vi "Two Color Calibration.vi"(7 "Calling VI Ref":refnum<vi>) -> ()   [LabVIEW 2016]
uses:
  <vilib>/Utility/miscctls.llb/LVPointTypeDef.ctl
  Hardware Configuration/Hardware Configuration Controls/Device Type.ctl
  Hardware Configuration/Hardware Configuration Controls/Device Function.ctl
  Two Color Cal Type Defs/Two Color Cal Notifier Type.ctl
  Two Color Cal Type Defs/Two Color Cal Actions.ctl
  Two Color Cal Type Defs/Two Color Last Used Parameters.ctl
  Orca Flash Capture Manager/SMS Analysis Interface/SMS Analysis Interface Type Defs/SMS Analysis Interface Connection Info.ctl
  Tools/TIFF Image Read and Write/ImageJ TIF Type Defs/TIF Write Image Information.ctl
  Device Library/Cameras/Camera Controls/Generic Camera Actions.ctl
  Laser Control/Laser Power Control/Laser Power Control Type Defs/Laser Power Ctrl Messenger Actions.ctl
  Device Library/Stages/Stages Controls/Stage Actions.ctl
  shell32.dll
panel:
  out "Transfer Error":bool
  in  "Auto Focus":bool
  in  "Auto Run":bool=TRUE
  out "File Close":errorcluster
  in  "Skip":bool
  in  "Run Capture":bool
  in  "Number of Y Steps":u16=10
  out "Current Y Step":u16
  out "Current X Step":u16
  in  "Number of X Steps":u16=10
  in  "Step Size (µm)":dbl=2.0
  in  "Start":bool
  in  "Quit":bool
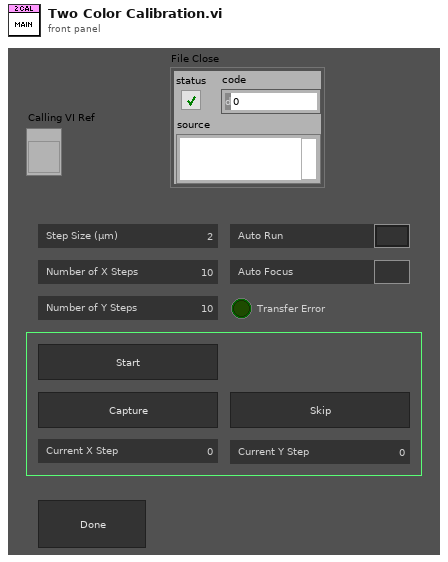
[diagram p1: front panel]
types:
  T1 = typedef "SMS Analysis Interface Connection Info.ctl" = cluster{"Remote IP":string, "Port":u16}
  T2 = typedef "Two Color Last Used Parameters.ctl" = cluster{"Step Size (um)":dbl, "No X Steps":u16, "No Y Steps":u16, "Auto Run":bool, "Auto Focus":bool}
  T3 = typedef "Device Function.ctl" = enum16{"Primary", "Secondary", "Overview", "Wide Field Drift Correction", "642 nm Excitation", "560 nm Excitation", "940 nm Excitation", "546 nm Excitation", "488 nm Excitation", "405 nm Excitation", "Objective Drift Correction", "4Pi Objective Lock", "Objective XY", "Objective Z", "Sample XY", "Sample Coarse Z", "Sample Z", "4Pi Lower", "4Pi Upper", "Mojo", "Adj Cavity", "Line Scanning", "Alert"}
  T4 = typedef "Device Type.ctl" = enum16{"AOTF", "Camera", "Deformable Mirror", "Laser", "Shutter", "Stage", "Waveform", "FPGA", "Email", "Filter Wheel"}
  T5 = typedef "Two Color Cal Actions.ctl" = enum16{"Idle", "Set File Name", "Open FIle", "Start Camera", "Laser On", "Auto Focus", "Capture", "Move XY", "Pause Scan", "Abort", "Send Image", "Quit"}
  T6 = typedef "Two Color Cal Notifier Type.ctl" = cluster{"Actions":T5, "X Steps":u16, "Y Steps":u16, "Save File Path":path, "Save File Ref":refnum<file>}
  T7 = enum16{"Always On", "Always Off", "Off While Running"}
  T8 = typedef "LVPointTypeDef.ctl" = cluster{"Horizontal":i16, "Vertical":i16}
  T9 = typedef "Generic Camera Actions.ctl" = enum16{"Status", "Live Preview", "Capture", "Abort", "Set Exposure Time (s)", "Get Exposure Time (s)", "Record Settings", "Binning", "Set ROI", "Get ROI", "Defect Correction On?", "Cooler On?", "Fan On?", "Quit"}
  T10 = typedef "TIF Write Image Information.ctl" = cluster{"Image Width (Pixels)":u32, "Image Height (Pixels)":u32, "Pixel Width (µm)":dbl, "Pixel Height (µm)":dbl, "Bits Per Sample (e.g. 16)":u32, "No. of Frames":u32, "No. of Slices":u32, "Time Step (sec)":dbl, "Z Step (µm)":dbl}
  T11 = typedef "Laser Power Ctrl Messenger Actions.ctl" = enum16{"All Active On", "All Off", "Adjust Power", "Line On/Off", "Get Status"}
  T12 = typedef "Stage Actions.ctl" = enum16{"Get Position", "MVR", "MOVE", "HALT", "ONTARGET", "ERROR", "REFERENCE", "INIT", "VELOCITY", "STATUS", "EXIT", "HOME", "ZEROPOS", "NANOPOS", "ANALOG", "QUIT"}
  T13 = enum32{"Invalid", "Standard", "Closed", "Hidden", "Minimized", "Maximized"}
  T14 = typedef "IMAQ Image.ctl" = refnum<image>
  T15 = typedef "Camera IMAQ Key Info.ctl" = cluster{"Frame":u32, "Sensor Height":i32, "Sensor Width":i32, "ROI Height":i32, "ROI Width":i32, "ROI Enable?":bool, "Bit per Pixel":u8}
  T16 = typedef "LVRectTypeDef.ctl" = cluster{"Left":i16, "Top":i16, "Right":i16, "Bottom":i16}
  T17 = typedef "LVBoundsTypeDef.ctl" = cluster{"Width":u32, "Height":u32}
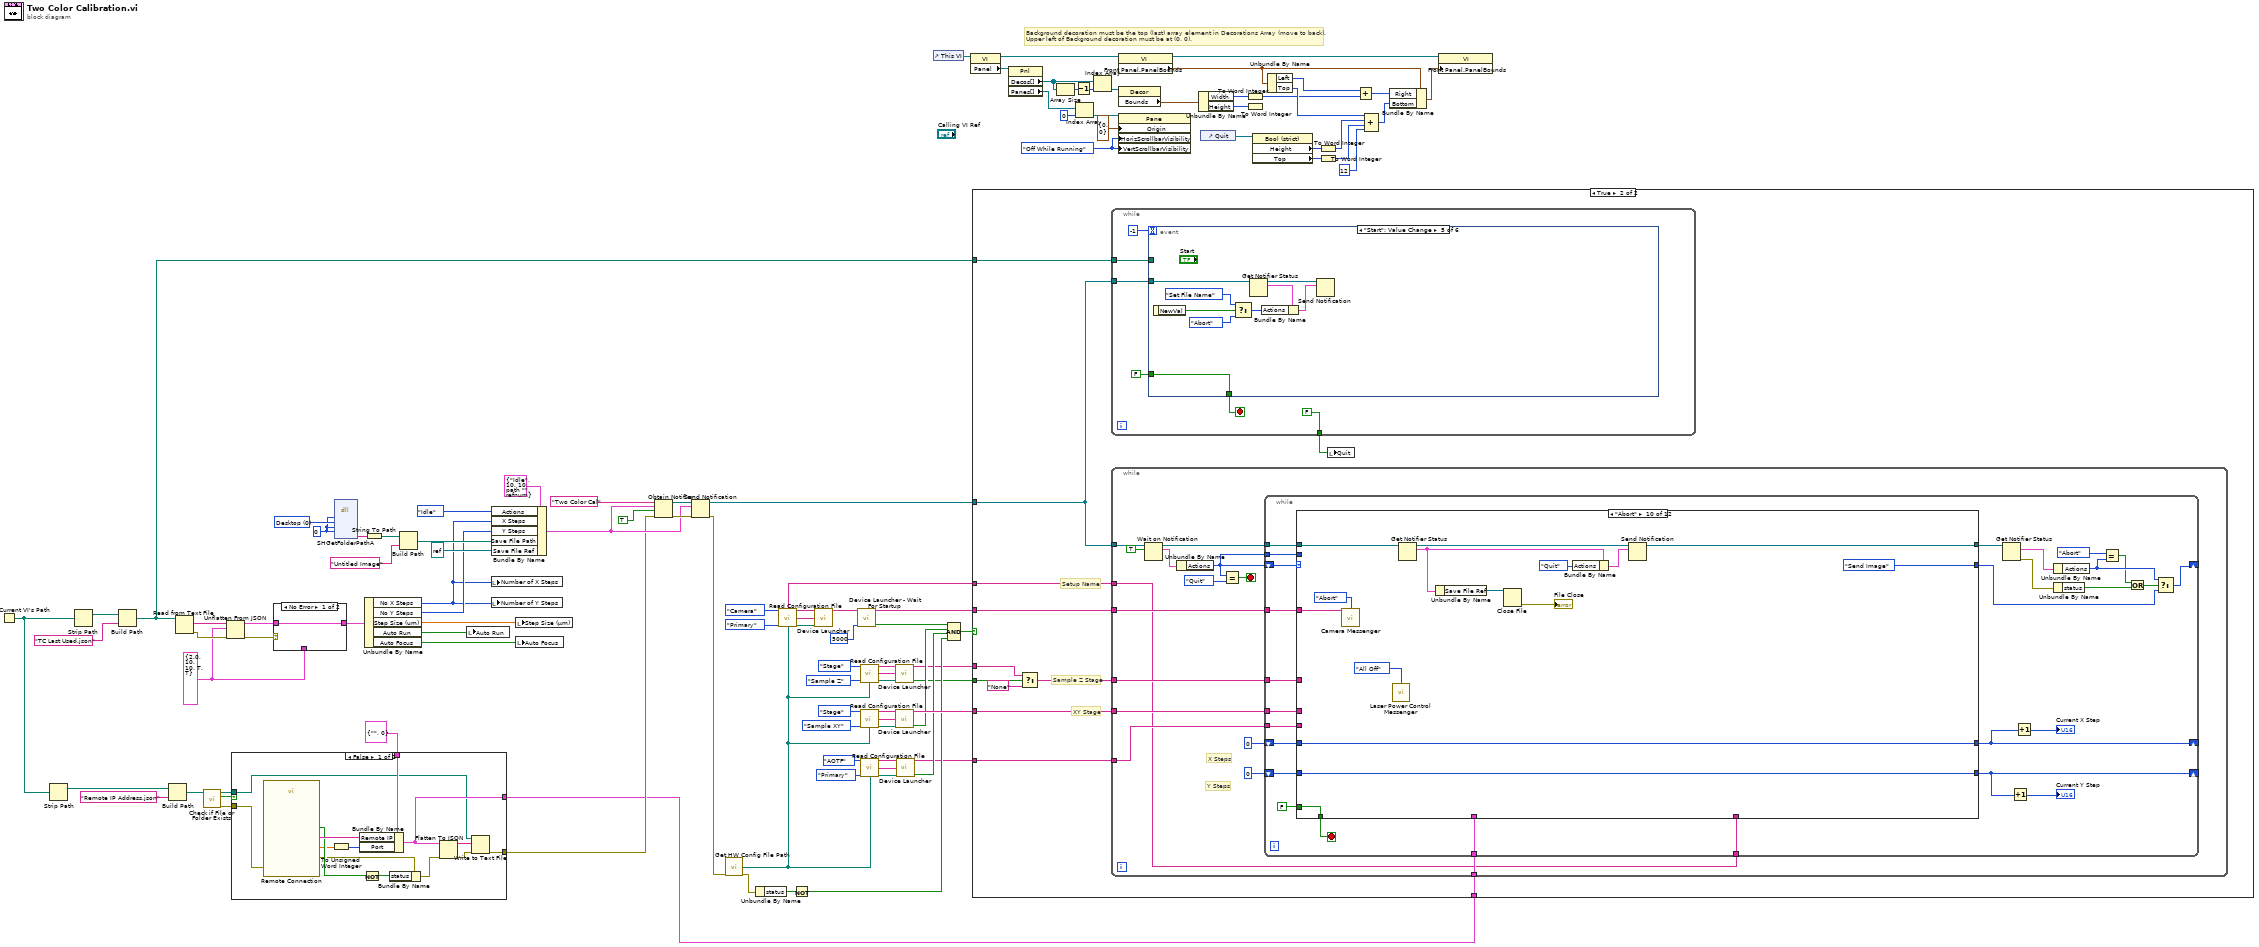
[diagram p0: block diagram]
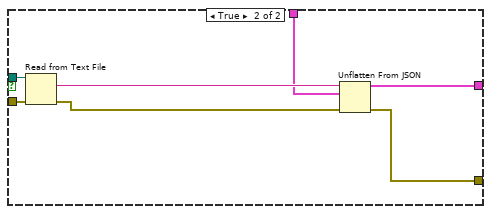
[diagram p2: hidden frame]
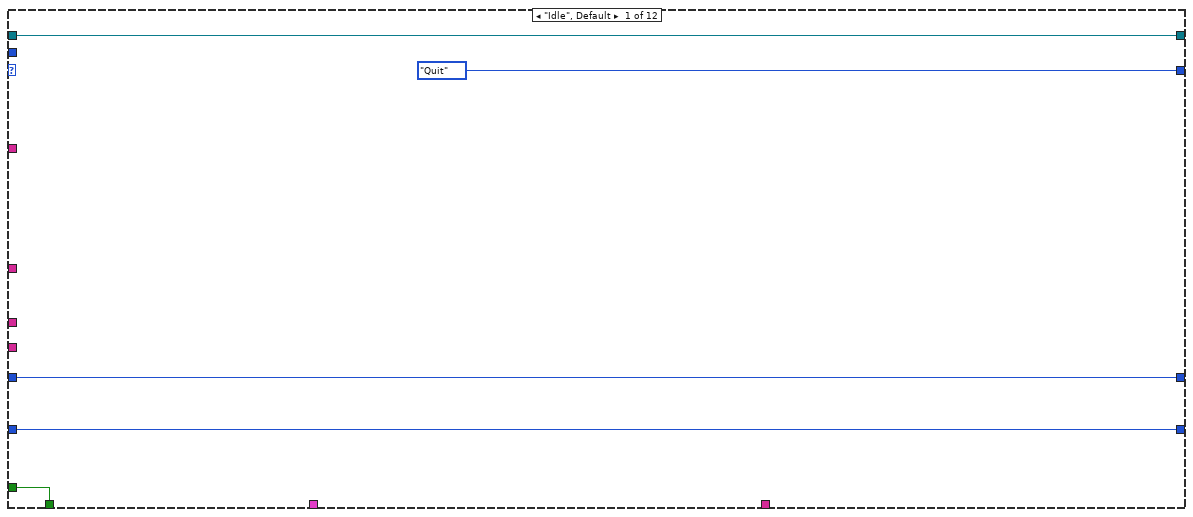
[diagram p5: hidden frame]
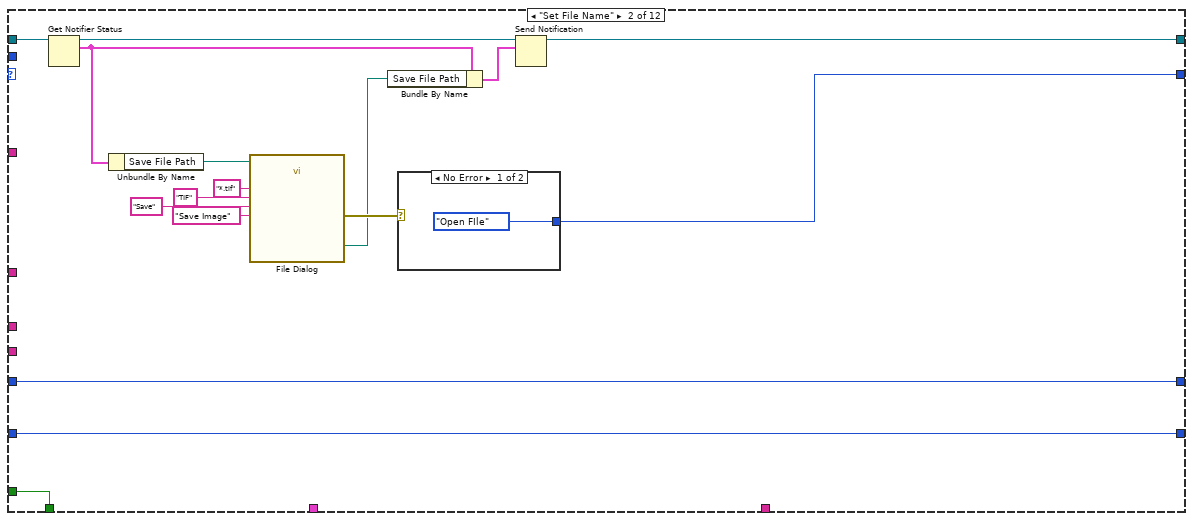
[diagram p6: hidden frame]
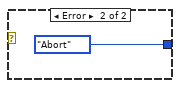
[diagram p7: hidden frame]
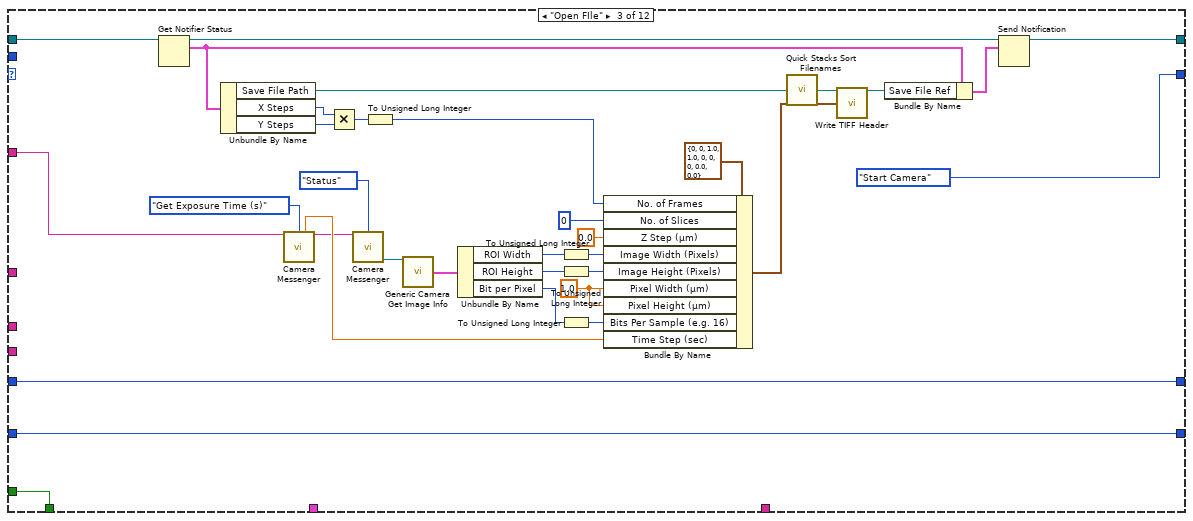
[diagram p8: hidden frame]
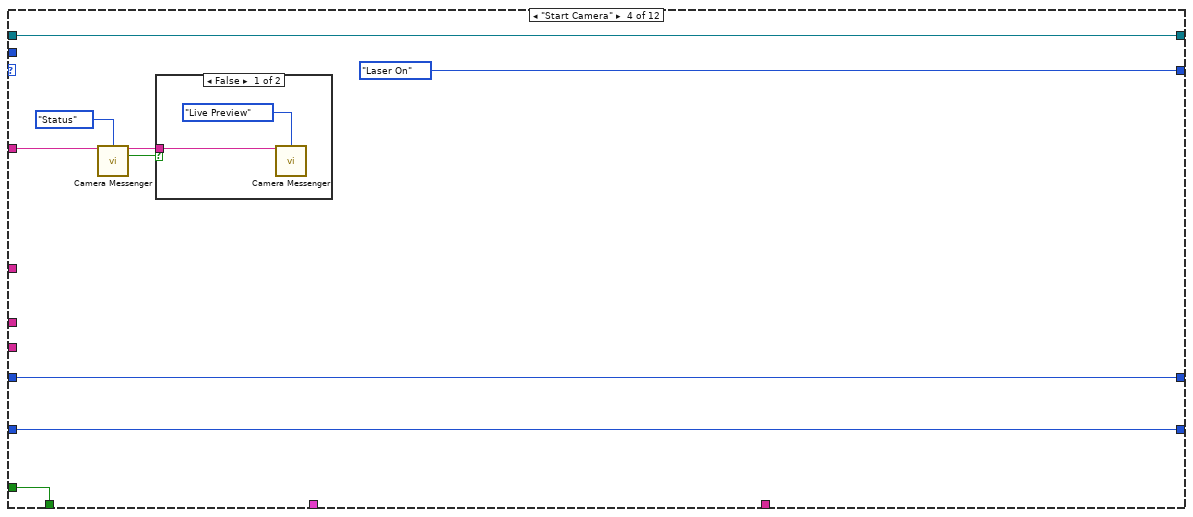
[diagram p9: hidden frame]
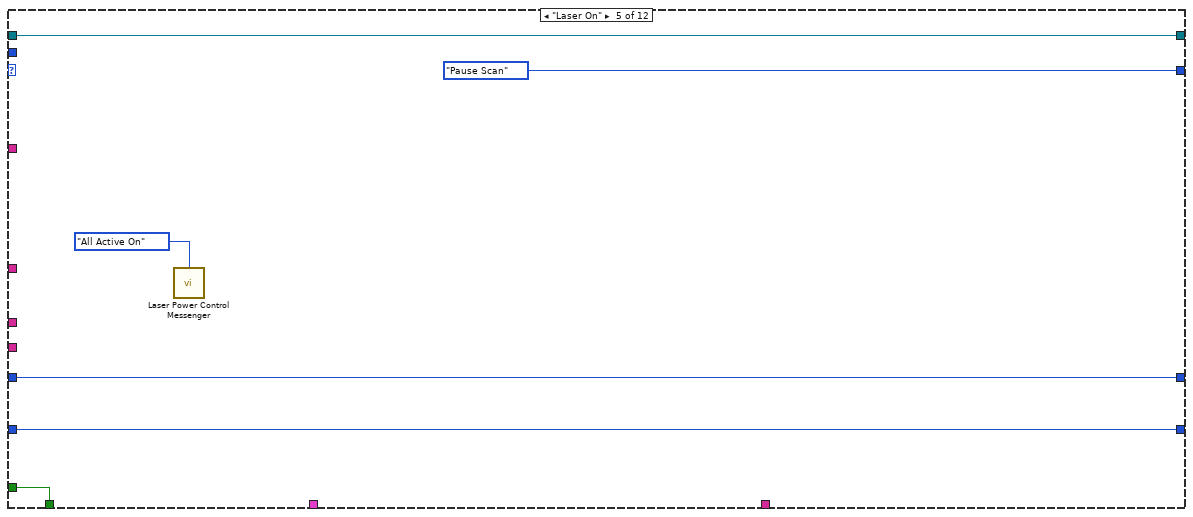
[diagram p11: hidden frame]
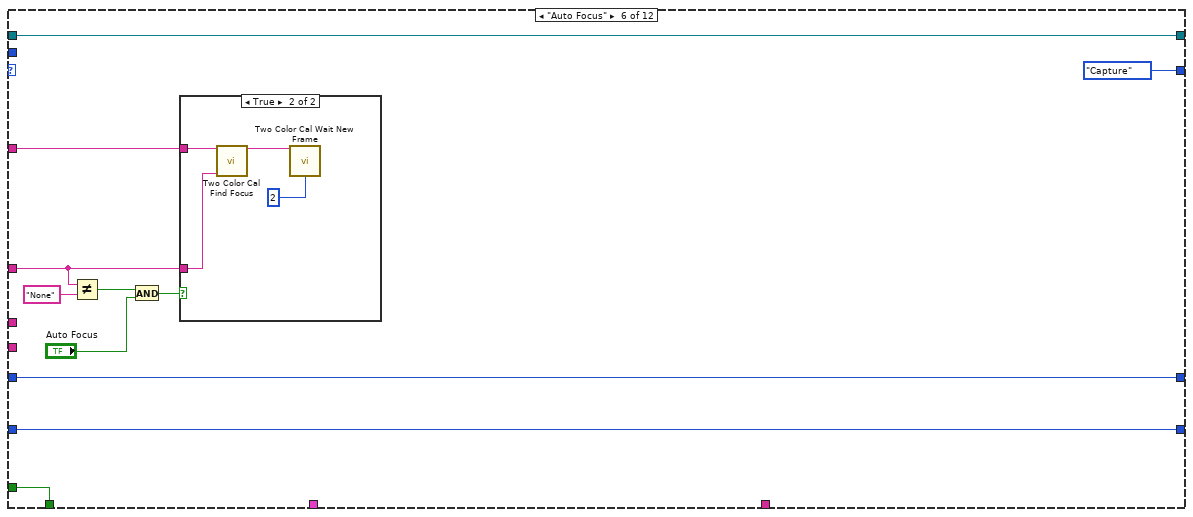
[diagram p12: hidden frame]
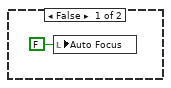
[diagram p13: hidden frame]
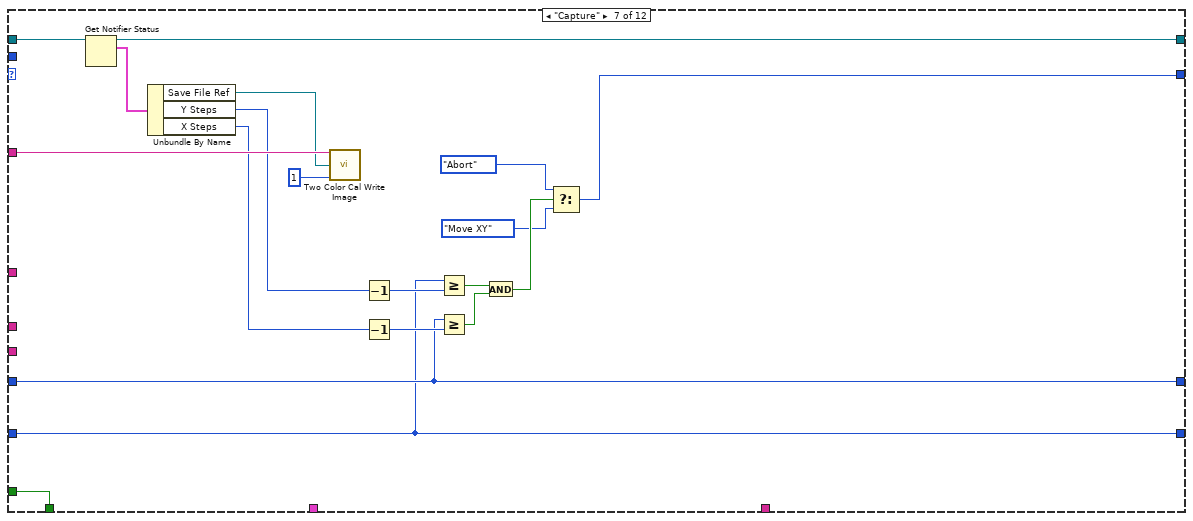
[diagram p14: hidden frame]
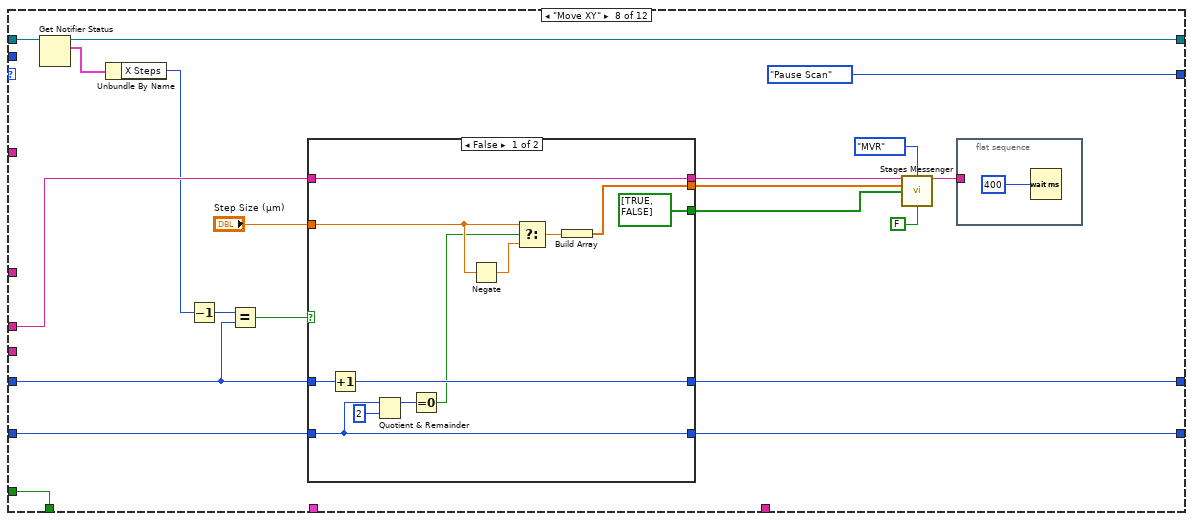
[diagram p15: hidden frame]
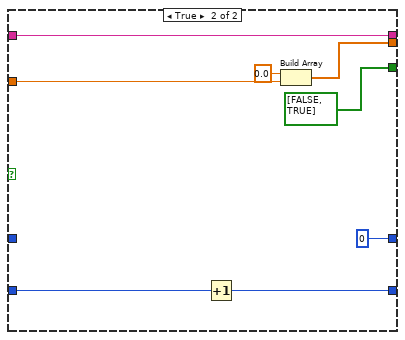
[diagram p16: hidden frame]
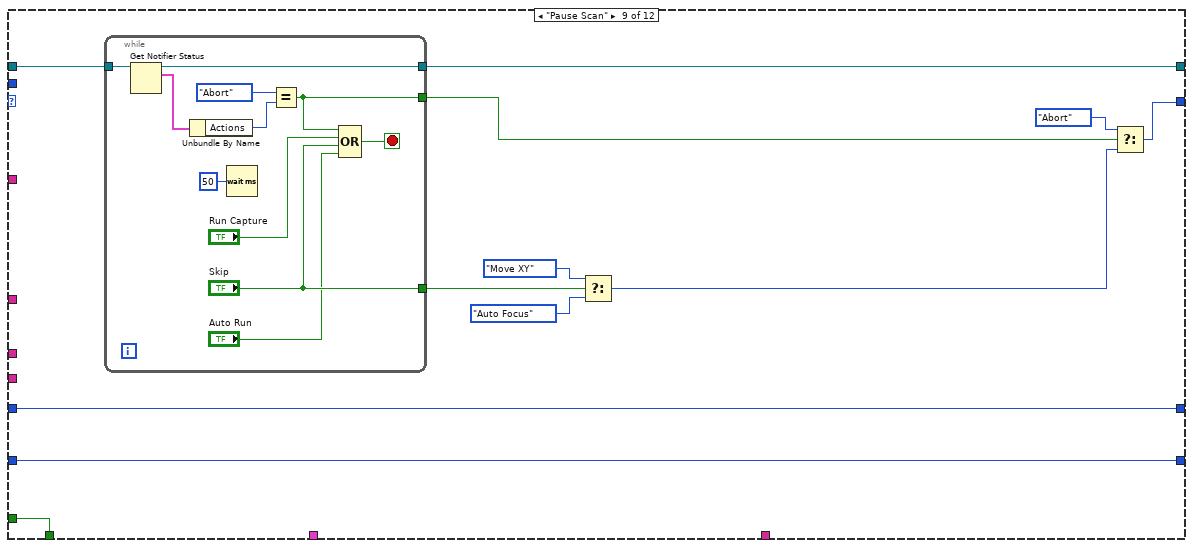
[diagram p17: hidden frame]
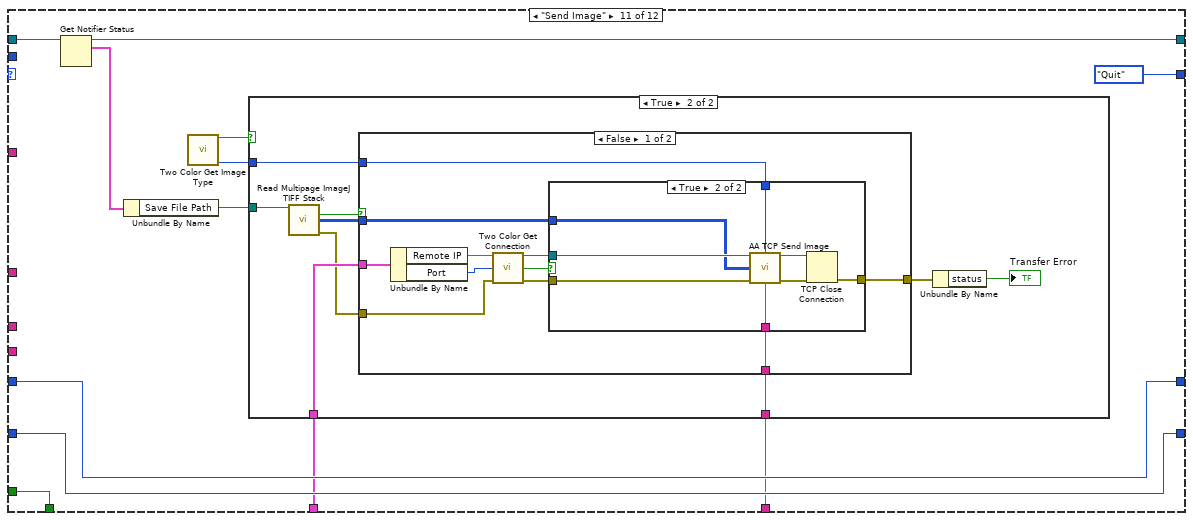
[diagram p18: hidden frame]
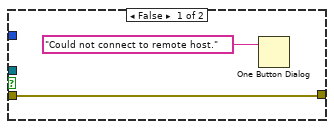
[diagram p20: hidden frame]
diagram:
  w19 = T2 {"Step Size (um)"=2.0, "No X Steps"=10, "No Y Steps"=10, "Auto Run"=TRUE, "Auto Focus"=TRUE} ("Last Used Parameters")
  w51 = 0 items=["Desktop"=0, "Personal Documents"=5, "AppData"=26, "Local AppData"=28, "Common AppData"=35, "Program Files"=38, "Program Files Common"=43, "Common Documents"=46] ("Requested Path")
  w50 = 0 ("HWND")
  w88 = T7."Off While Running" ("Vertical Scrollbar Visibility")
  # "Background decoration must be the top (last) array element in Decorations Array (move to back).\nUpper left of Background decoration must be at (0, 0)."
  n1 = Current VI's Path() -> (path=w4:path)
  n2 = Strip Path(path=w4) -> (stripped path=w10:path)  [unwired: 1 out]
  n3 = Strip Path(path=w4) -> (stripped path=w25:path)  [unwired: 1 out]
  n4 = Build Path(base path=w25, name or relative path="TC Last Used.json") -> (appended path=w12:path)
  n5 = Build Path(base path=w10, name or relative path="Remote IP Address.json" ("name (unnamed)")) -> (appended path=w7:path)
  n6 = Read from Text File(file (use dialog)=w12) -> (text=w23:string, error out=w22:errorcluster)  [unwired: 3 in, 2 out]
  n7 = call <vilib>:"Check if File or Folder Exists.vi"("path"=w7) -> ("error out"=w5:errorcluster, "file or folder exists?"=w8:bool, "dup path"=w9:path)  [unwired: 8 in]
  n8 = Unflatten From JSON(JSON string=w23, type and defaults=w19, error in (no error)=w22) -> (value=w20:T2, error out=w21:errorcluster)  [unwired: 4 in]
  n9 = case shown="False" w8 {
    tunnel: w9 -> [w112 w124]
    tunnel: [w118 w123] -> w2
    tunnel: T1 {"Remote IP"="", "Port"=0} ("Connection Data") -> [w119 w122]
    tunnel: [w113 w120] -> w3
    tunnel: w5 -> [w110 w121]
    frame False {
      n10 = call "Remote Connection"("error in (no error)"=w110) -> ("Port"=w107:dbl, "IP Address"=w111:string, "OK"=w109:bool, "error out"=w108:errorcluster)  [unwired: 15 in]
      n11 = To Unsigned Word Integer(number=w107) -> (unsigned 16bit integer=w106:u16)
      n12 = Bundle By Name(cluster=w119, "Remote IP"=w111, "Port"=w106) -> (w118:T1)
      n13 = Not(x=w109) -> (.not. x?=w115:bool)
      n14 = Bundle By Name(cluster=w108, "status"=w115) -> (w114:errorcluster)
      n15 = Flatten To JSON(anything=w118, error in (no error)=w114) -> (JSON string=w117:string, 11:w116:errorcluster)  [unwired: 1 in]
      n16 = Write to Text File(file (use dialog)=w112, text=w117, error in=w116) -> (error out=w113:errorcluster)  [unwired: 1 in, 2 out]
    }
    frame True {
      n17 = Read from Text File(file (use dialog)=w124, error in=w121) -> (text=w126:string, error out=w125:errorcluster)  [unwired: 2 in, 2 out]
      n18 = Unflatten From JSON(JSON string=w126, type and defaults=w122, error in (no error)=w125) -> (value=w123:T1, error out=w120:errorcluster)  [unwired: 4 in]
    }
  }
  n19 = case shown="No Error" w21 {
    tunnel: w20 -> [w127 _]
    tunnel: [w127 w128] -> w18
    tunnel: w19 -> [_ w128]
    frame No Error {
    }
    frame Error {
    }
  }
  n20 = dll-call lib="shell32.dll" fn="SHGetFolderPathA"("HWND"=w50, "nFolder"=w51, "hToken"=w50, "dwFlags"=w50) -> ("pszPath"=w49:string)  [unwired: 9 in, 2 out]
  n21 = Unbundle By Name(w18) -> ("No X Steps"=w13:u16, "No Y Steps"=w14:u16, "Step Size (um)"=w15:dbl, "Auto Run"=w17:bool, "Auto Focus"=w16:bool)
  n22 = String To Path(string=w49) -> (path=w47:path)
  n23 = Build Path(base path=w47, name or relative path="Untitled Image") -> (appended path=w44:path)
  n24 = local write "Auto Run"(w17) -> ()
  n25 = Bundle By Name(cluster=T6 {"Actions"=enum."Idle", "X Steps"=10, "Y Steps"=10, "Save File Path"=path "", "Save File Ref"=refnum} ("Two Color Notifier Type"), "Actions"=Two_Color_Cal_Actions."Idle", "X Steps"=w13, "Y Steps"=w14, "Save File Path"=w44, "Save File Ref"=refnum<file> refnum) -> (w42:T6)
  n26 = local write "Number of X Steps"(w13) -> ()
  n27 = local write "Number of Y Steps"(w13) -> ()
  n28 = local write "Step Size (µm)"(w15) -> ()
  n29 = local write "Auto Focus"(w16) -> ()
  n30 = Obtain Notifier(name (unnamed)="Two Color Cal", notification data type=w42, create if not found? (T)=TRUE, error in (no error)=w3) -> (notifier out=w74:refnum<notifier>, error out=w73:errorcluster)  [unwired: 1 out]
  n31 = Send Notification(notification=w42, notifier=w74, error in (no error)=w73) -> (notifier out=w72:refnum<notifier>, error out=w71:errorcluster)
  n32 = call "Get HW Config File Path.vi"("Error"=w71) -> ("File Path"=w28:path, "Error"=w57:errorcluster)  [unwired: 13 in]
  n33 = Unbundle By Name(w57) -> ("status"=w56:bool)
  n34 = call "Read Configuration File.vi"("Device Type"=Device_Type."Camera", "Device Function"=Device_Function."Primary", "Config File Path"=w28) -> ("Configuration Name"=w1:string, "Unique Notifier Name"=w68:string, "Device Ports/IDs/Channels"=w70:string[], "Device Engine Path"=w69:path)  [unwired: 9 in]
  n35 = Not(x=w56) -> (.not. x?=w35:bool)
  n36 = call "Device Launcher.vi"("Notifier Name"=w68, "Device Ports/IDs/Channels"=w70, "Device Engine Path"=w69) -> ("Notifier Name"=w66:string)  [unwired: 11 in, 1 out]
  n37 = call "Device Launcher - Wait For Startup.vi"("Notifier Name"=w66, "Wait Time (ms)"=5000) -> ("Notifier Name (Dup)"=w52:string, "Running?"=w55:bool)  [unwired: 12 in]
  n38 = call "Read Configuration File.vi"("Device Type"=Device_Type."Stage", "Device Function"=Device_Function."Sample Z", "Config File Path"=w28) -> ("Unique Notifier Name"=w31:string, "Device Ports/IDs/Channels"=w33:string[], "Device Engine Path"=w32:path)  [unwired: 9 in, 1 out]
  n39 = call "Read Configuration File.vi"("Device Type"=Device_Type."Stage", "Device Function"=Device_Function."Sample XY", "Config File Path"=w28) -> ("Unique Notifier Name"=w61:string, "Device Ports/IDs/Channels"=w59:string[], "Device Engine Path"=w60:path)  [unwired: 9 in, 1 out]
  n40 = call "Read Configuration File.vi"("Device Type"=Device_Type."AOTF", "Device Function"=Device_Function."Primary", "Config File Path"=w28) -> ("Unique Notifier Name"=w41:string, "Device Ports/IDs/Channels"=w39:string[], "Device Engine Path"=w40:path)  [unwired: 9 in, 1 out]
  n41 = call "Device Launcher.vi"("Notifier Name"=w31, "Device Ports/IDs/Channels"=w33, "Device Engine Path"=w32) -> ("Notifier Name"=w27:string, "Running?"=w26:bool)  [unwired: 11 in]
  n42 = call "Device Launcher.vi"("Notifier Name"=w61, "Device Ports/IDs/Channels"=w59, "Device Engine Path"=w60) -> ("Notifier Name"=w58:string, "Running?"=w54:bool)  [unwired: 11 in]
  n43 = call "Device Launcher.vi"("Notifier Name"=w41, "Device Ports/IDs/Channels"=w39, "Device Engine Path"=w40) -> ("Notifier Name"=w34:string, "Running?"=w36:bool)  [unwired: 11 in]
  n44 = control-ref of="This VI"() -> (w80:refnum<vi>)
  n45 = Compound Arithmetic op=AND(w55, w54, w36, w35) -> (w53:bool)
  n46 = property class="VI"(reference=w80) -> (reference out=w89:refnum<vi>, "Panel"=w81:refnum<vi>)  [unwired: 1 in, 1 out]
  n47 = case shown="True" w53 {
    tunnel: w72 -> [_ w139]
    tunnel: w58 -> [_ w138]
    tunnel: w52 -> [_ w137]
    tunnel: w34 -> [_ w136]
    tunnel: w27 -> [_ w134]
    tunnel: w26 -> [_ w135]
    tunnel: w12 -> [_ w131]
    tunnel: w2 -> [_ w130]
    tunnel: w1 -> [_ w129]
    frame False {
    }
    frame True {
      # "Setup Name"
      # "Sample Z Stage"
      # "XY Stage"
      n48 = Select(t=w134, s=w135, f="None") -> (s? t:f=w132:string)
      n49 = while {
        tunnel: [FALSE] -> w140
        tunnel: w139 -> [w424]
        tunnel: w131 -> [w423]
        stop <- w426 stop-if-true
        n50 = event shown="[4] \"Start\": Value Change" {
          selector: _ -> [_ _ _ _ _ _]
          dyn-events: _ -> [_ _ _ _ _ _]
          timeout: -1 -> [_ _ _ _ _ _]
          tunnel: FALSE -> [w429 w433 w441 w448 w457 _]
          tunnel: [w429 w433 w441 w448 w457 w473] -> w426
          tunnel: w424 -> [_ _ w440 w447 w455 w471]
          tunnel: w423 -> [_ _ _ _ _ w459]
          event Timeout {
            n51 = event-data() -> ()  [unwired: 1 in, 1 out]
          }
          event Application Instance Close? {
            n52 = event-data() -> ()  [unwired: 1 in, 1 out]
            n53 = control-ref of="This VI"() -> (w430:refnum<vi>)
            n54 = invoke class="VI" method="FP.Open"(reference=w430, "Activate"=TRUE ("Activate?"), "State"=T13."Standard") -> ()  [unwired: 2 in, 5 out]
            n55 = event-data("Discard?"=TRUE) -> ()  [unwired: 1 in, 1 out]
          }
          event "Number of X Steps": Value Change {
            n56 = event-data() -> ("NewVal"=w435:u16)  [unwired: 1 in]
            n57 = Get Notifier Status(notifier=w440) -> (notifier out=w437:refnum<notifier>, current notification=w439:T6)  [unwired: 1 in, 3 out]
            n58 = Bundle By Name(cluster=w439, "Actions"=Two_Color_Cal_Actions."Idle", "X Steps"=w435) -> (w436:T6)
            n59 = Send Notification(notification=w436, notifier=w437) -> ()  [unwired: 1 in, 2 out]
          }
          event "Number of Y Steps": Value Change {
            n60 = event-data() -> ("NewVal"=w442:u16)  [unwired: 1 in]
            n61 = Get Notifier Status(notifier=w447) -> (notifier out=w444:refnum<notifier>, current notification=w446:T6)  [unwired: 1 in, 3 out]
            n62 = Bundle By Name(cluster=w446, "Actions"=Two_Color_Cal_Actions."Idle", "Y Steps"=w442) -> (w443:T6)
            n63 = Send Notification(notification=w443, notifier=w444) -> ()  [unwired: 1 in, 2 out]
          }
          event "Start": Value Change {
            n64 = event-data() -> ("NewVal"=w452:bool)  [unwired: 1 in]
            n65 = Select(t=Two_Color_Cal_Actions."Set File Name" ("Actions"), s=w452, f=Two_Color_Cal_Actions."Abort" ("Actions")) -> (s? t:f=w449:T5)
            n66 = Get Notifier Status(notifier=w455) -> (notifier out=w456:refnum<notifier>, current notification=w454:T6)  [unwired: 1 in, 3 out]
            n67 = Bundle By Name(cluster=w454, "Actions"=w449) -> (w453:T6)
            n68 = Send Notification(notification=w453, notifier=w456) -> ()  [unwired: 1 in, 2 out]
          }
          event "Quit": Value Change {
            n69 = event-data() -> ("NewVal"=w473:bool)  [unwired: 1 in]
            n70 = Get Notifier Status(notifier=w471) -> (notifier out=w472:refnum<notifier>, current notification=w468:T6)  [unwired: 1 in, 3 out]
            n71 = Bundle By Name(cluster=w468, "Actions"=Two_Color_Cal_Actions."Quit") -> (w469:T6)
            n72 = Send Notification(notification=w469, notifier=w472) -> ()  [unwired: 1 in, 2 out]
            n73 = Unbundle By Name(w468) -> ("X Steps"=w463:u16, "Y Steps"=w462:u16)
            n74 = local read "Step Size (µm)"() -> (w465:dbl)
            n75 = local read "Auto Focus"() -> (w466:bool)
            n76 = local read "Auto Run"() -> (w467:bool)
            n77 = Bundle By Name(cluster=T2 {"Step Size (um)"=0.0, "No X Steps"=0, "No Y Steps"=0, "Auto Run"=FALSE, "Auto Focus"=FALSE} ("Last Used Parameters"), "No X Steps"=w463, "No Y Steps"=w462, "Step Size (um)"=w465, "Auto Run"=w467, "Auto Focus"=w466) -> (w461:T2)
            n78 = Flatten To JSON(anything=w461) -> (JSON string=w460:string, 11:w458:errorcluster)  [unwired: 2 in]
            n79 = Write to Text File(file (use dialog)=w459, text=w460, error in=w458) -> ()  [unwired: 1 in, 3 out]
          }
        }
      }
      n80 = while {
        tunnel: w138 -> [w150]
        tunnel: w139 -> [w155]
        tunnel: w137 -> [w147]
        tunnel: w136 -> [w144]
        tunnel: w132 -> [w143]
        tunnel: w130 -> [w142]
        tunnel: w129 -> [w141]
        stop <- w152 stop-if-true
        # "Y Steps"
        # "X Steps"
        n81 = Wait on Notification(notifier=w155, ignore previous (F)=TRUE) -> (notifier out=w151:refnum<notifier>, notification=w146:T6)  [unwired: 2 in, 2 out]
        n82 = Unbundle By Name(w146) -> ("Actions"=w145:T5)
        n83 = Equal?(x=w145, y=Two_Color_Cal_Actions."Quit") -> (x = y?=w152:bool)
        n84 = while {
          tunnel: w151 -> [w182]
          tunnel: w150 -> [w178]
          tunnel: w145 -> [w177]
          shift-right: [w161] -> _
          shift-left: w145 -> [w181]
          shift-right: [w174] -> _
          shift-left: u16 0 -> [w176]
          shift-right: [w173] -> _
          shift-left: u16 0 -> [w175]
          tunnel: w147 -> [w172]
          tunnel: w144 -> [w171]
          tunnel: w143 -> [w158]
          tunnel: w142 -> [w157]
          tunnel: w141 -> [w156]
          stop <- w179 stop-if-true
          n85 = case shown="\"Abort\"" w181 {
            tunnel: w182 -> [w183 w200 w236 w242 w255 w267 w279 w297 w338 w367 w380 w415]
            tunnel: FALSE -> [w187 w203 w239 w248 w256 w266 w291 w310 w344 w370 w382 _]
            tunnel: [w187 w203 w239 w248 w256 w266 w291 w310 w344 w370 w382 TRUE] -> w179
            tunnel: w178 -> [_ _ _ _ _ _ _ w309 _ _ _ _]
            tunnel: w177 -> [_ _ _ _ _ _ _ _ _ _ _ w420]
            tunnel: [Two_Color_Cal_Actions."Quit" ("y") w189 Two_Color_Cal_Actions."Start Camera" ("y") Two_Color_Cal_Actions."Laser On" ("y") Two_Color_Cal_Actions."Pause Scan" ("y") Two_Color_Cal_Actions."Capture" ("y") w289 Two_Color_Cal_Actions."Pause Scan" ("y") w333 Two_Color_Cal_Actions."Send Image" ("y") Two_Color_Cal_Actions."Quit" ("y") Two_Color_Cal_Actions."Quit" ("y")] -> w162
            tunnel: w176 -> [w185 w202 w238 w247 w253 w261 w283 w294 w343 w369 w375 w418]
            tunnel: w175 -> [w184 w201 w237 w246 w252 w260 w282 w301 w342 w368 w376 w417]
            tunnel: [w185 w202 w238 w247 w253 w261 w283 w307 w343 w369 w375 w418] -> w174
            tunnel: [w184 w201 w237 w246 w252 w260 w282 w300 w342 w368 w376 w417] -> w173
            tunnel: w172 -> [_ _ w206 w243 _ w262 w281 _ _ w364 _ _]
            tunnel: [w183 w188 w234 w242 w255 w267 w274 w296 w337 w361 w378 w415] -> w163
            tunnel: w171 -> [_ _ _ _ _ _ _ _ _ _ _ _]
            tunnel: w158 -> [_ _ _ _ _ w263 _ _ _ _ _ _]
            tunnel: w157 -> [_ _ _ _ _ _ _ _ _ _ w374 _]
            tunnel: w156 -> [_ _ _ _ _ _ _ _ _ _ w373 _]
            frame "Idle", Default {
            }
            frame "Set File Name" {
              n86 = Get Notifier Status(notifier=w200) -> (notifier out=w199:refnum<notifier>, current notification=w198:T6)  [unwired: 1 in, 3 out]
              n87 = Unbundle By Name(w198) -> ("Save File Path"=w196:path)
              n88 = call "File Dialog"("start path"=w196, "prompt"="Save Image", "button label"="Save", "pattern (all files)"="*.tif", "pattern label"="TIF") -> ("selected path"=w190:path, "error out"=w195:errorcluster)  [unwired: 7 in, 2 out]
              n89 = Bundle By Name(cluster=w198, "Save File Path"=w190) -> (w197:T6)
              n90 = case shown="No Error" w195 {
                tunnel: [Two_Color_Cal_Actions."Open FIle" ("y") Two_Color_Cal_Actions."Abort" ("y")] -> w189
                frame No Error {
                }
                frame Error {
                }
              }
              n91 = Send Notification(notification=w197, notifier=w199) -> (notifier out=w188:refnum<notifier>)  [unwired: 1 in, 1 out]
            }
            frame "Open FIle" {
              w227 = 1.0 ("Pixel Width (µm)")
              n92 = Get Notifier Status(notifier=w236) -> (notifier out=w208:refnum<notifier>, current notification=w210:T6)  [unwired: 1 in, 3 out]
              n93 = Unbundle By Name(w210) -> ("Save File Path"=w214:path, "X Steps"=w218:u16, "Y Steps"=w217:u16)
              n94 = call "Camera Messenger.vi"("Notifier Name"=w206, "General Camera Actions"=Generic_Camera_Actions."Get Exposure Time (s)") -> ("Current Exposure Time (s)"=w231:dbl, "Notifier Name Dup"=w230:string)  [unwired: 8 in, 4 out]
              n95 = Multiply(x=w218, y=w217) -> (x*y=w216:u16)
              n96 = call "Camera Messenger.vi"("Notifier Name"=w230, "General Camera Actions"=Generic_Camera_Actions."Status") -> ("Image Ref"=w222:T14)  [unwired: 8 in, 5 out]
              n97 = To Unsigned Long Integer(number=w216) -> (unsigned 32bit integer=w215:u32)
              n98 = call "Generic Camera Get Image Info.vi"("Image Ref"=w222) -> ("Camera Image Info"=w223:T15)  [unwired: 14 in]
              n99 = Unbundle By Name(w223) -> ("ROI Width"=w224:i32, "ROI Height"=w225:i32, "Bit per Pixel"=w226:u8)
              n100 = To Unsigned Long Integer(number=w224) -> (unsigned 32bit integer=w212:u32)
              n101 = To Unsigned Long Integer(number=w225) -> (unsigned 32bit integer=w211:u32)
              n102 = To Unsigned Long Integer(number=w226) -> (unsigned 32bit integer=w213:u32)
              n103 = Bundle By Name(cluster=T10 {"Image Width (Pixels)"=0, "Image Height (Pixels)"=0, "Pixel Width (µm)"=1.0, "Pixel Height (µm)"=1.0, "Bits Per Sample (e.g. 16)"=0, "No. of Frames"=0, "No. of Slices"=0, "Time Step (sec)"=0.0, "Z Step (µm)"=0.0} ("Image Info"), "No. of Frames"=w215, "No. of Slices"=u32 0, "Z Step (µm)"=0.0, "Image Width (Pixels)"=w212, "Image Height (Pixels)"=w211, "Pixel Width (µm)"=w227, "Pixel Height (µm)"=w227, "Bits Per Sample (e.g. 16)"=w213, "Time Step (sec)"=w231) -> (w221:T10)
              n104 = call "Quick Stacks Sort Filenames.vi"("Requested File Path"=w214) -> ("Resulting File Path"=w219:path)  [unwired: 14 in]
              n105 = call "Write TIFF Header.vi"("File Path"=w219, "Image Info"=w221) -> ("File Ref"=w209:refnum<file>)  [unwired: 11 in, 2 out]
              n106 = Bundle By Name(cluster=w210, "Save File Ref"=w209) -> (w207:T6)
              n107 = Send Notification(notification=w207, notifier=w208) -> (notifier out=w234:refnum<notifier>)  [unwired: 1 in, 1 out]
            }
            frame "Start Camera" {
              n108 = call "Camera Messenger.vi"("Notifier Name"=w243, "General Camera Actions"=Generic_Camera_Actions."Status") -> ("Notifier Name Dup"=w244:string, "Running?"=w240:bool)  [unwired: 8 in, 4 out]
              n109 = case shown="False" w240 {
                tunnel: w244 -> [w250 _]
                frame False {
                  n110 = call "Camera Messenger.vi"("Notifier Name"=w250, "General Camera Actions"=Generic_Camera_Actions."Live Preview") -> ()  [unwired: 8 in, 6 out]
                }
                frame True {
                }
              }
            }
            frame "Laser On" {
              n111 = call "Laser Power Control Messenger.vi"("Power Ctrl Actions"=Laser_Power_Ctrl_Messenger_Actions."All Active On") -> ()  [unwired: 13 in, 2 out]
            }
            frame "Auto Focus" {
              n112 = Not Equal?(x=w263, y="None") -> (x != y?=w259:bool)
              n113 = And(x=w259, y="Auto Focus") -> (x .and. y?=w257:bool)
              n114 = case shown="True" w257 {
                tunnel: w263 -> [_ w271]
                tunnel: w262 -> [_ w272]
                frame False {
                  n115 = local write "Auto Focus"(FALSE ("Auto Focus")) -> ()
                }
                frame True {
                  n116 = call "Two Color Cal Find Focus.vi"("Camera Notifier Name"=w272, "Z Stage Notifier Name"=w271) -> ("Camera Notifier (Dup)"=w269:string)  [unwired: 13 in]
                  n117 = call "Two Color Cal Wait New Frame.vi"("Notifier Name"=w269, "Frames to Wait"=u32 2) -> ()  [unwired: 13 in, 1 out]
                }
              }
            }
            frame "Capture" {
              n118 = Get Notifier Status(notifier=w279) -> (notifier out=w274:refnum<notifier>, current notification=w278:T6)  [unwired: 1 in, 3 out]
              n119 = Unbundle By Name(w278) -> ("Save File Ref"=w277:refnum<file>, "Y Steps"=w276:u16, "X Steps"=w275:u16)
              n120 = call "Two Color Cal Write Image.vi"("Notifier Name"=w281, "Write File Ref"=w277, "Num of Frames"=u16 1) -> ()  [unwired: 13 in]
              n121 = Decrement(x=w276) -> (x-1=w288:u16)
              n122 = Decrement(x=w275) -> (x-1=w287:u16)
              n123 = Greater Or Equal?(x=w282, y=w288) -> (x >= y?=w286:bool)
              n124 = Greater Or Equal?(x=w283, y=w287) -> (x >= y?=w285:bool)
              n125 = And(x=w286, y=w285) -> (x .and. y?=w284:bool)
              n126 = Select(t=Two_Color_Cal_Actions."Abort" ("y"), s=w284, f=Two_Color_Cal_Actions."Move XY" ("y")) -> (s? t:f=w289:T5)
            }
            frame "Move XY" {
              n127 = Get Notifier Status(notifier=w297) -> (notifier out=w296:refnum<notifier>, current notification=w298:T6)  [unwired: 1 in, 3 out]
              n128 = Unbundle By Name(w298) -> ("X Steps"=w295:u16)
              n129 = Decrement(x=w295) -> (x-1=w293:u16)
              n130 = Equal?(x=w293, y=w294) -> (x = y?=w292:bool)
              n131 = case shown="False" w292 {
                tunnel: w309 -> [w323 w330]
                tunnel: "Step Size (µm)" -> [w318 w328]
                tunnel: [w324 u16 0] -> w307
                tunnel: w294 -> [w320 _]
                tunnel: [w323 w330] -> w304
                tunnel: [w322 w331] -> w303
                tunnel: [bool[] [TRUE, FALSE] ("Axis") bool[] [FALSE, TRUE] ("Axis")] -> w302
                tunnel: w301 -> [w316 w327]
                tunnel: [w316 w326] -> w300
                frame False {
                  n132 = Increment(x=w320) -> (x+1=w324:u16)
                  n133 = Quotient & Remainder(x=w316, y=u16 2) -> (x-y*floor(x/y)=w314:u16)  [unwired: 1 out]
                  n134 = Equal To 0?(x=w314) -> (x = 0?=w313:bool)
                  n135 = Negate(x=w318) -> (-x=w317:dbl)
                  n136 = Select(t=w318, s=w313, f=w317) -> (s? t:f=w319:dbl)
                  n137 = Build Array(w319) -> (w322:dbl[])
                }
                frame True {
                  n138 = Increment(x=w327) -> (x+1=w326:u16)
                  n139 = Build Array(0.0 ("element"), w328) -> (w331:dbl[])
                }
              }
              n140 = call "Stages Messenger.vi"("Stage Notifier Name"=w304, "Actions"=Stage_Actions."MVR", "Setpoint"=w303, "Axis"=w302, "Exit While Busy?"=FALSE) -> ("Stage Notifier Name (Dup)"=w299:string)  [unwired: 7 in, 3 out]
              n141 = flat-sequence {
                tunnel: w299 -> [_]
                frame #0 {
                  n142 = Wait (ms)(milliseconds to wait=u32 400 ("Stage Delay")) -> ()  [unwired: 1 out]
                }
              }
            }
            frame "Pause Scan" {
              n143 = while {
                tunnel: ["Skip"] -> w341
                tunnel: w338 -> [w354]
                tunnel: [w353] -> w337
                tunnel: [w347] -> w336
                stop <- w350 stop-if-true
                n144 = Get Notifier Status(notifier=w354) -> (notifier out=w353:refnum<notifier>, current notification=w355:T6)  [unwired: 1 in, 3 out]
                n145 = Unbundle By Name(w355) -> ("Actions"=w351:T5)
                n146 = Wait (ms)(milliseconds to wait=u32 50) -> ()  [unwired: 1 out]
                n147 = Equal?(x=Two_Color_Cal_Actions."Abort", y=w351) -> (x = y?=w347:bool)
                n148 = Compound Arithmetic op=OR(w347, "Run Capture", "Skip", "Auto Run") -> (w350:bool)
              }
              n149 = Select(t=Two_Color_Cal_Actions."Move XY" ("y"), s=w341, f=Two_Color_Cal_Actions."Auto Focus" ("y")) -> (s? t:f=w334:T5)
              n150 = Select(t=Two_Color_Cal_Actions."Abort" ("x"), s=w336, f=w334) -> (s? t:f=w333:T5)
            }
            frame "Abort" {
              n151 = call "Camera Messenger.vi"("Notifier Name"=w364, "General Camera Actions"=Generic_Camera_Actions."Abort") -> ()  [unwired: 8 in, 6 out]
              n152 = call "Laser Power Control Messenger.vi"("Power Ctrl Actions"=Laser_Power_Ctrl_Messenger_Actions."All Off") -> ()  [unwired: 13 in, 2 out]
              n153 = Get Notifier Status(notifier=w367) -> (notifier out=w362:refnum<notifier>, current notification=w360:T6)  [unwired: 1 in, 3 out]
              n154 = Unbundle By Name(w360) -> ("Save File Ref"=w366:refnum<file>)
              n155 = Close File(refnum=w366) -> (error out=→"File Close":errorcluster)  [unwired: 1 in, 1 out]
              n156 = Bundle By Name(cluster=w360, "Actions"=Two_Color_Cal_Actions."Quit") -> (w358:T6)
              n157 = Send Notification(notification=w358, notifier=w362) -> (notifier out=w361:refnum<notifier>)  [unwired: 1 in, 1 out]
            }
            frame "Send Image" {
              n158 = Get Notifier Status(notifier=w380) -> (notifier out=w378:refnum<notifier>, current notification=w379:T6)  [unwired: 1 in, 3 out]
              n159 = Unbundle By Name(w379) -> ("Save File Path"=w377:path)
              n160 = call "Two Color Get Image Type.vi"() -> ("Canceled?"=w372:bool, "Spooler Code"=w371:u8)  [unwired: 14 in]
              n161 = case shown="True" w372 {
                tunnel: w377 -> [_ w391]
                tunnel: w374 -> [_ w388]
                tunnel: w373 -> [_ w384]
                tunnel: w371 -> [_ w383]
                frame False {
                }
                frame True {
                  n162 = call "Read Multipage ImageJ TIFF Stack.vi"("ImageJ Tif Path"=w391) -> ("U8 Image?"=w390:bool, "U16 Stack"=w389:u16[][][], "Error Out"=w387:errorcluster)  [unwired: 10 in, 2 out]
                  n163 = case shown="False" w390 {
                    tunnel: w389 -> [w399 _]
                    tunnel: w388 -> [w402 _]
                    tunnel: w387 -> [w395 w413]
                    tunnel: [w394 w413] -> w386
                    tunnel: w384 -> [w393 _]
                    tunnel: w383 -> [w392 _]
                    frame False {
                      n164 = Unbundle By Name(w402) -> ("Remote IP"=w401:string, "Port"=w397:u16)
                      n165 = call "Two Color Get Connection.vi"("Remote IP"=w401, "Port"=w397, "Error In"=w395) -> ("Connection ID"=w400:refnum<k5>, "Connected?"=w398:bool, "Error Out"=w396:errorcluster)  [unwired: 10 in]
                      n166 = case shown="True" w398 {
                        tunnel: w400 -> [_ w412]
                        tunnel: w399 -> [_ w411]
                        tunnel: w396 -> [w403 w408]
                        tunnel: [w403 w407] -> w394
                        tunnel: w393 -> [_ w406]
                        tunnel: w392 -> [_ w405]
                        frame False {
                          n167 = One Button Dialog(message="Could not connect to remote host.") -> ()  [unwired: 1 in, 1 out]
                        }
                        frame True {
                          n168 = call "AA TCP Send Image.vi"("Connection ID"=w412, "Spooler Code"=w405, "Image Stack (U16)"=w411, "Error In"=w408, "Setup Name"=w406) -> ("Connection ID Out"=w410:refnum<k5>, "Error Out"=w409:errorcluster)  [unwired: 8 in, 1 out]
                          n169 = TCP Close Connection(connection ID=w410, error in (no error)=w409) -> (error out=w407:errorcluster)  [unwired: 1 in, 1 out]
                        }
                      }
                    }
                    frame True {
                      n170 = One Button Dialog(message="8 bit images not supported for automatic transfer.") -> ()  [unwired: 1 in, 1 out]
                    }
                  }
                  n171 = Unbundle By Name(w386) -> ("status"=→"Transfer Error":bool)
                }
              }
            }
            frame "Quit" {
              n172 = local write "Start"(FALSE ("Start")) -> ()
              n173 = case shown="\"Quit\"" w420 {
                tunnel: w415 -> [_ w422]
                frame Default {
                }
                frame "Quit" {
                  n174 = Release Notifier(notifier=w422) -> ()  [unwired: 2 in, 3 out]
                }
              }
            }
          }
          n175 = Get Notifier Status(notifier=w163) -> (current notification=w164:T6, error out=w165:errorcluster)  [unwired: 1 in, 3 out]
          n176 = Increment(x=w173) -> (x+1=→"Current Y Step":u16)
          n177 = Increment(x=w174) -> (x+1=→"Current X Step":u16)
          n178 = Unbundle By Name(w164) -> ("Actions"=w170:T5)
          n179 = Unbundle By Name(w165) -> ("status"=w167:bool)
          n180 = Equal?(x=Two_Color_Cal_Actions."Abort", y=w170) -> (x = y?=w168:bool)
          n181 = Or(x=w168, y=w167) -> (x .or. y?=w169:bool)
          n182 = Select(t=w170, s=w169, f=w162) -> (s? t:f=w161:T5)
        }
      }
      n183 = local write "Quit"(w140) -> ()
    }
  }
  n184 = property class="Pnl"(reference=w81) -> ("Decos[]"=w79:refnum<vi>[], "Panes[]"=w85:refnum<vi>[])  [unwired: 1 in, 2 out]
  n185 = Array Size(array=w79) -> (size(s)=w77:i32)
  n186 = Decrement(x=w77) -> (x-1=w78:i32)
  n187 = Index Array(array=w85, index=0) -> (element=w84:refnum<vi>)
  n188 = Index Array(array=w79, index=w78) -> (element=w87:refnum<vi>)
  n189 = property class="VI"(reference=w89) -> (reference out=w91:refnum<vi>, "Front Panel.PanelBounds"=w92:T16)  [unwired: 1 in, 1 out]
  n190 = property class="Decor"(reference=w87) -> ("Bounds"=w90:T17)  [unwired: 1 in, 2 out]
  n191 = property class="Pane"(reference=w84, "Origin"=T8 {"Horizontal"=0, "Vertical"=0}, "HorizScrollbarVisibility"=w88, "VertScrollbarVisibility"=w88) -> ()  [unwired: 1 in, 2 out]
  n192 = Unbundle By Name(w90) -> ("Width"=w95:u32, "Height"=w98:u32)
  n193 = control-ref of="Quit"() -> (w82:refnum<vi>)
  n194 = To Word Integer(number=w95) -> (16bit integer=w97:i16)
  n195 = To Word Integer(number=w98) -> ()  [unwired: 1 out]
  n196 = property class="Bool (strict)"(reference=w82) -> ("Height"=w100:u32, "Top"=w101:i32)  [unwired: 1 in, 2 out]
  n197 = Unbundle By Name(w92) -> ("Left"=w94:i16, "Top"=w105:i16)
  n198 = To Word Integer(number=w100) -> (16bit integer=w103:i16)
  n199 = To Word Integer(number=w101) -> (16bit integer=w104:i16)
  n200 = Add(x=w94, y=w97) -> (x+y=w96:i16)
  n201 = Compound Arithmetic op=ADD(w105, w103, w104, i16 12 ("y")) -> (w99:i16)
  n202 = Bundle By Name(cluster=w92, "Right"=w96, "Bottom"=w99) -> (w93:T16)
  n203 = property class="VI"(reference=w91, "Front Panel.PanelBounds"=w93) -> ()  [unwired: 1 in, 2 out]
